vi "Network Streams Chat Window Launcher Server.vi"() -> ()   [LabVIEW 2020]
uses:
  Chat Window/Chat Window.lvclass
  C:/Program Files/National Instruments/LabVIEW 2026/vi.lib/ActorFramework/Actor/Actor.lvclass
  Chat Window/Chat Window.lvclass/Chat Window.ctl
  Protocols/Network Stream Strategy/Netowrk Stream Listener/Network Stream Listener.lvclass
  C:/Data/1_Projects/network-endpoint-actors/Source/Abstract Classes/Message Stream/Message Stream.lvclass
  <vilib>/ActorFramework/Actor/Actor.lvclass
panel:
  in  "Listener Name":string="Bob"
  out "error out":errorcluster
  # "This VI launches two instances of a chat window actor.  The two chat windows launch nested endpoints, which connect via a Network Stream mesage stream.\n\n1.  (Optional)  Specify the IP address for this machine, and the names of the two stream endpoints\n2.  Run this VI.\n3.  Stop the application by closing either chat window.\n\nAF_Debug_Trace is set to TRUE in this project, so you can follow the action with the Desktop Execution Trace Toolkit."
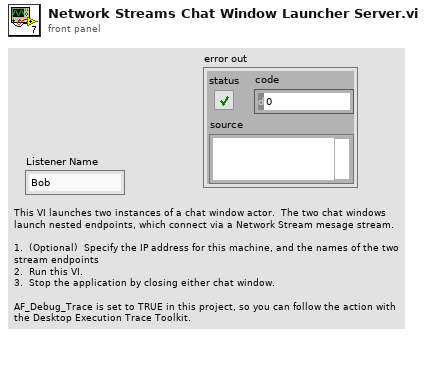
[diagram p1: front panel]
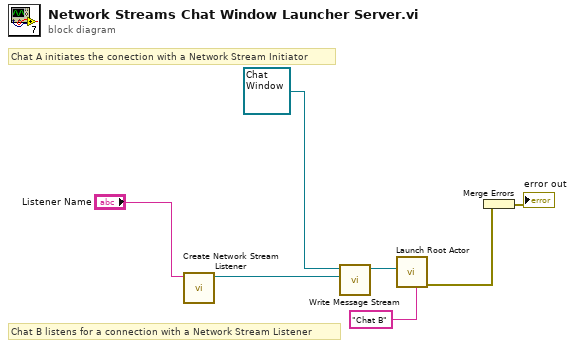
[diagram p0: block diagram]
diagram:
  # "Chat B listens for a connection with a Network Stream Listener"
  # "Chat A initiates the conection with a Network Stream Initiator"
  n1 = call "Create Network Stream Listener.vi"("Name"="Listener Name") -> ("Network Stream Listener"=w2:refnum<class "Network Stream Listener.lvclass">)  [unwired: 10 in]
  n2 = call "Write Message Stream.vi"("Message Stream"=w2, "Chat Window in"=refnum<class "Chat Window.lvclass"> refnum) -> ("Chat Window out"=w3:refnum<class "Chat Window.lvclass">)  [unwired: 9 in]
  n3 = call <vilib>:"Launch Root Actor.vi"("Debug Alias"="Chat B", "Actor"=w3) -> ("error out"=w5:errorcluster)  [unwired: 8 in, 1 out]
  n4 = Merge Errors(w5) -> (→"error out":errorcluster)
